vi "Sim_Validate_Setpoints.vi"(7 "Settings":T1={"UI Update Interval (ms)"=200, "Max dt (s)"=1.0, "Initial SOC (%)"=50.0, "Rest Voltage (V)"=12.0, "Ambient Temperature (degC)"=25.0, "Voltage Time Constant (s)"=5.0, "Current Time Constant (s)"=1.0, "Thermal Time Constant (s)"=120.0, "Heating Coefficient (degC/s per A^2)"=0.002, "SOC Speed Factor"=1.0, "Charge Complete SOC (%)"=100.0, "Discharge Complete SOC (%)"=0.0, "Max Voltage Limit (V)"=15.0, "Max Current Limit (A)"=10.0, "Max Temperature Limit (degC)"=45.0, "Max C-Rate (1/h)"=5.0, "Max Duration (min)"=600.0, "History Length (samples)"=3000, "Inject E-Stop"=FALSE, "Inject Overvoltage"=FALSE, "Inject Overcurrent"=FALSE, "Inject Overtemperature"=FALSE}, 8 "Duration (min)":dbl, 9 "C-Rate (1/h)":dbl, 10 "Current (A)":dbl, 11 "Voltage (V)":dbl) -> (2 "Message":string, 3 "Valid?":bool)   [LabVIEW 2019]
doc: "Validates the setpoints of the selected operation before Start. Each value must be finite, greater than 0 and not above its limit in Simulation Settings (DEMO ONLY). NaN and Inf fail automatically because every comparison with them is FALSE. Message names the FIRST failing value in the order Voltage, Current, C-Rate, Duration."
uses:
  Sim_Settings.ctl
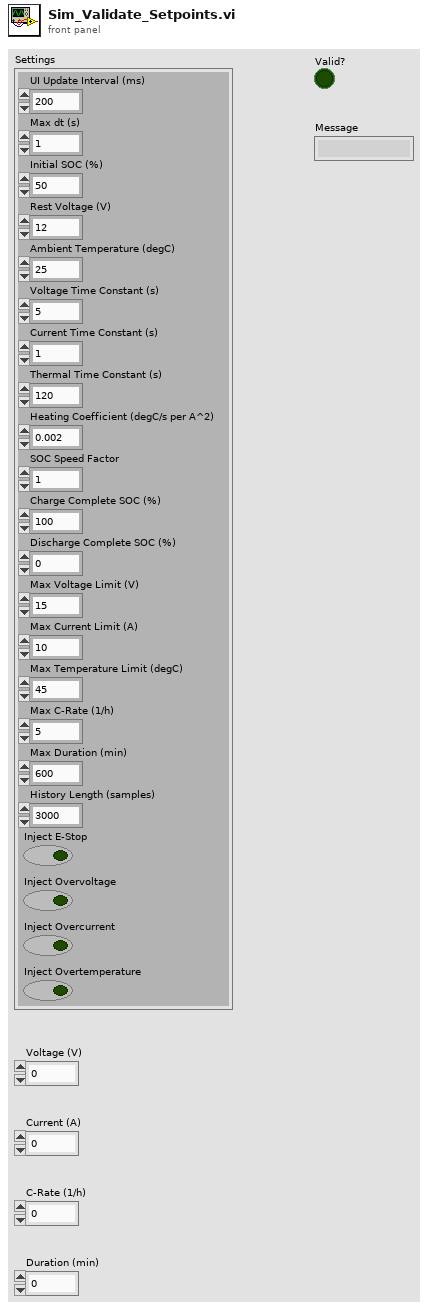
[diagram p1: front panel]
types:
  T1 = typedef "Sim_Settings.ctl" = cluster{"UI Update Interval (ms)":i32, "Max dt (s)":dbl, "Initial SOC (%)":dbl, "Rest Voltage (V)":dbl, "Ambient Temperature (degC)":dbl, "Voltage Time Constant (s)":dbl, "Current Time Constant (s)":dbl, "Thermal Time Constant (s)":dbl, "Heating Coefficient (degC/s per A^2)":dbl, "SOC Speed Factor":dbl, "Charge Complete SOC (%)":dbl, "Discharge Complete SOC (%)":dbl, "Max Voltage Limit (V)":dbl, "Max Current Limit (A)":dbl, "Max Temperature Limit (degC)":dbl, "Max C-Rate (1/h)":dbl, "Max Duration (min)":dbl, "History Length (samples)":i32, "Inject E-Stop":bool, "Inject Overvoltage":bool, "Inject Overcurrent":bool, "Inject Overtemperature":bool}
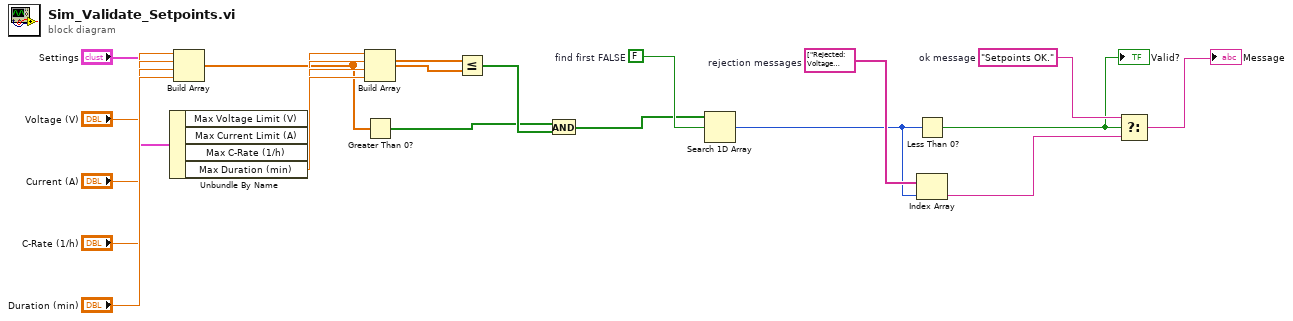
[diagram p0: block diagram]
diagram:
  w20 = "Setpoints OK."  # ok message
  w18 = string[] ["Rejected: Voltage setpoint must be > 0 and <= Max Voltage Limit (Simulation Settings).", "Rejected: Current setpoint must be > 0 and <= Max Current Limit (Simulation Settings).", "Rejected: C-Rate must be > 0 and <= Max C-Rate (Simulation Settings).", "Rejected: Duration must be > 0 and <= Max Duration (Simulation Settings)."]  # rejection messages
  w15 = FALSE  # find first FALSE
  n1 = Unbundle By Name("Settings") -> ("Max Voltage Limit (V)"=w7:dbl, "Max Current Limit (A)"=w8:dbl, "Max C-Rate (1/h)"=w9:dbl, "Max Duration (min)"=w10:dbl)
  n2 = Build Array("Voltage (V)", "Current (A)", "C-Rate (1/h)", "Duration (min)") -> (w6:dbl[])
  n3 = Build Array(w7, w8, w9, w10) -> (w11:dbl[])
  n4 = Greater Than 0?(x=w6) -> (x > 0?=w12:bool[])
  n5 = Less Or Equal?(x=w6, y=w11) -> (x <= y?=w13:bool[])
  n6 = And(x=w12, y=w13) -> (x .and. y?=w14:bool[])
  n7 = Search 1D Array(1D array=w14, element=w15) -> (index of element=w16:i32)  [unwired: 1 in]
  n8 = Less Than 0?(x=w16) -> (x < 0?=w17:bool)
  "Valid?" <- w17
  n9 = Index Array(array=w18, index=w16) -> (element=w19:string)
  n10 = Select(t=w20, s=w17, f=w19) -> (s? t:f=→"Message":string)
